vi "Write Loop.vi"(8 "error in (no error)":errorcluster caption="에러 입력(에러 없음)", 11 "TCP Socket 입력":refnum<class "TCP Socket.lvclass">) -> (0 "error out":errorcluster caption="에러 출력", 3 "TCP Socket 출력":refnum<class "TCP Socket.lvclass">)   [LabVIEW 2023, in "TCP Socket.lvclass"]
uses:
  TCP Socket.lvclass
  TCP Socket.lvclass/TCP Socket.ctl
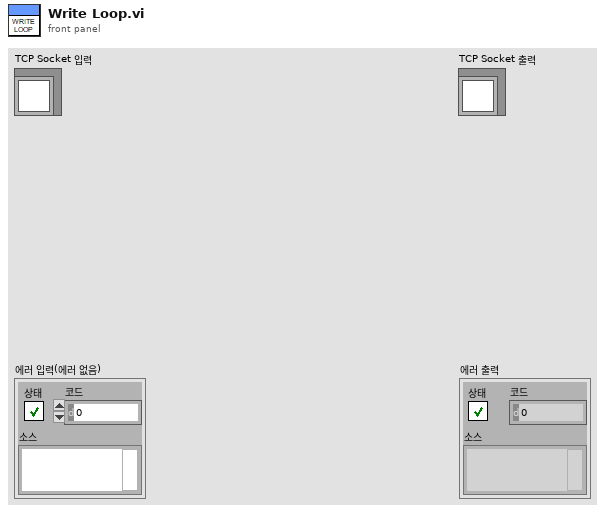
[diagram p1: front panel]
types:
  T1 = enum16{"big-endian, network order", "native, host order", "little-endian"}
  T2 = cluster{"Reader Q":refnum<queue>, "Writer Q":refnum<queue>}
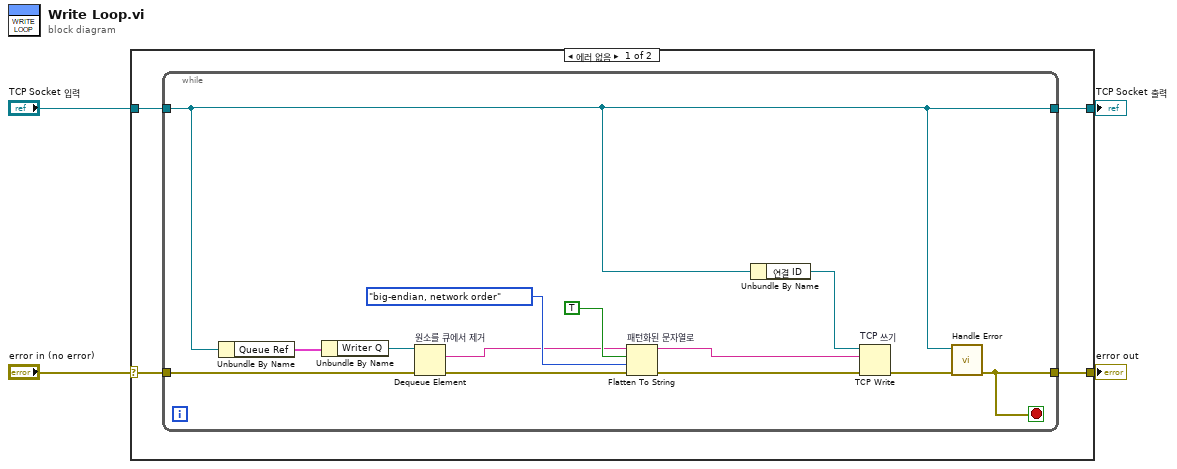
[diagram p0: block diagram]
diagram:
  n1 = case shown="에러 없음" "error in (no error)" {
    selector: "error in (no error)" -> [w8 w23]
    tunnel: [w5 w23] -> w3
    tunnel: [w6 w22] -> w1
    tunnel: "TCP Socket 입력" -> [w7 w22]
    frame No Error {
      n2 = while {
        tunnel: w8 -> [w21]
        tunnel: w7 -> [w15]
        tunnel: [w15] -> w6
        tunnel: [w16] -> w5
        stop <- w16 stop-if-true
        n3 = Unbundle By Name(w15) -> ("Queue Ref"=w20:T2)
        n4 = Unbundle By Name(w20) -> ("Writer Q"=w19:refnum<queue>)
        n5 = Dequeue Element "원소를 큐에서 제거"(queue=w19, error in (no error)=w21) -> (element=w12:string, error out=w10:errorcluster)  [unwired: 1 in, 2 out]
        n6 = Flatten To String "패턴화된 문자열로"(anything=w12, prepend array or string size? (T)=TRUE ("배열 또는 문자열 크기를 앞에 추가? (참)"), byte order (0:big-endian, network order)=T1."big-endian, network order" ("바이트 순서(0:big-endian, network order)"), error in (no error)=w10) -> (data string=w11:string, error out=w9:errorcluster)  [unwired: 1 out]
        n7 = Unbundle By Name(w15) -> ("연결 ID"=w18:refnum<k5>)
        n8 = TCP Write "TCP 쓰기"(connection ID=w18, data in=w11, error in (no error)=w9) -> (error out=w17:errorcluster)  [unwired: 1 in, 2 out]
        n9 = call "Handle Error.vi"("error in (no error)"=w17, "TCP Socket 입력"=w15) -> ("error out"=w16:errorcluster)  [unwired: 8 in, 1 out]
      }
    }
    frame Error {
    }
  }
  "error out" <- w3
  "TCP Socket 출력" <- w1
